vi "GUI_Bella_LaserTable.vi"() -> ()   [LabVIEW 2020]
uses:
  Shared/GUI_Template/GUI_master/tcp_new_data_event.ctl
  Shared/GUI_Template/GUI_master/tcp new data cluster.ctl
  <vilib>/vision/Image Controls.llb/IMAQ Image.ctl
  <vilib>/ErrorRing/Error Ring.xnode
panel:
  in  "Color 8":u32(colorbox) caption="Color"
  in  "Color 7":u32(colorbox) caption="Color"
  in  "Color 6":u32(colorbox)
  in  "Color 5":u32(colorbox) caption="Color"
  in  "Color 4":u32(colorbox) caption="Color"
  in  "Color 3":u32(colorbox) caption="Color"
  in  "Color 2":u32(colorbox) caption="Color"
  in  "Color1":u32(colorbox) caption="Color"
  in  "Color":u32(colorbox)
  in  "size3Y":dbl=280.0 caption="Size Y" min=0.0 max=0.0
  in  "analysis::6":bool caption="Blank Button"
  in  "meancounts::6":dbl=0.001 caption="MeanCounts" min=0.0 max=999999999.0 format="%_4f"
  in  "meancounts::8":dbl=0.001 caption="MeanCounts" min=0.0 max=999999999.0 format="%_4f"
  in  "analysis::8":bool caption="Blank Button"
  in  "size8Y":dbl=125.0 caption="Size Y" min=0.0 max=0.0
  in  "size1Y":dbl=70.0 caption="Size Y" min=0.0 max=0.0
  out "Display8":T1(plugin-control) caption="M1 Cam"
  in  "Target.X::8":dbl=0.001 caption="X" min=0.0 max=2000.0
  in  "Target.Y::8":dbl=0.001 caption="Y" min=0.0 max=2000.0
  in  "size8X":dbl=170.0 caption="Size X" min=0.0 max=0.0
  out "Display7":T1(plugin-control) caption="M1 Cam"
  in  "Target.X::7":dbl=0.001 caption="X" min=0.0 max=2000.0
  in  "Target.Y::7":dbl=0.001 caption="Y" min=0.0 max=2000.0
  in  "size7":dbl=210.0 caption="Size" min=0.0 max=0.0
  out "Display6":T1(plugin-control) caption="M1 Cam"
  in  "Target.X::6":dbl=0.001 caption="X" min=0.0 max=2000.0
  in  "Target.Y::6":dbl=0.001 caption="Y" min=0.0 max=2000.0
  in  "size6":dbl=20.0 caption="Size" min=0.0 max=0.0
  out "error out":errorcluster
  in  "GUIdevice 7":string="CAM-1BL-DM" caption="CAMERA 7"
  in  "GUIdevice 6":string="CAM-LT-Amp3Leak" caption="CAMERA 6"
  in  "GUIdevice 8":string="CAM-1BL-ShotControl" caption="CAMERA 8"
  out "image::7":T1(plugin-control) caption="M1 Cam"
  out "image::8":T1(plugin-control) caption="M1 Cam"
  in  "centroidx::6":dbl=0.001 caption="X" min=0.0 max=0.0
  in  "centroidy::7":dbl=0.001 caption="Y" min=0.0 max=0.0
  in  "centroidx::7":dbl=0.001 caption="X" min=0.0 max=0.0
  in  "exposure::7":dbl=0.001 caption="Exposure" min=3.8e-05 max=1.0 format="%_4p"
  in  "trigger::7":bool caption="Blank Button"
  in  "centroidy::6":dbl=0.001 caption="Y" min=0.0 max=0.0
  in  "exposure::8":dbl=0.001 caption="Exposure" min=3.8e-05 max=1.0 format="%_4p"
  in  "trigger::8":bool caption="Blank Button"
  in  "centroidy::8":dbl=0.001 caption="Y" min=0.0 max=0.0
  in  "centroidx::8":dbl=0.001 caption="X" min=0.0 max=0.0
  in  "exposure::6":dbl=0.001 caption="Exposure" min=3.8e-05 max=1.0 format="%_4p"
  in  "trigger::6":bool caption="Blank Button"
  in  "image::6":T1(plugin-control) caption="M1 Cam"
  in  "roi::6":bool caption="Blank Button"
  in  "roi::7":bool caption="Blank Button"
  in  "roi::8":bool caption="Blank Button"
  out "Display5":T1(plugin-control) caption="M1 Cam"
  in  "Target.X::5":dbl=0.001 caption="X" min=0.0 max=2000.0
  in  "Target.Y::5":dbl=0.001 caption="Y" min=0.0 max=2000.0
  in  "size5":dbl=20.0 caption="Size" min=0.0 max=0.0
  out "Display4":T1(plugin-control) caption="M1 Cam"
  in  "Target.X::4":dbl=0.001 caption="X" min=0.0 max=2000.0
  in  "Target.Y::4":dbl=0.001 caption="Y" min=0.0 max=2000.0
  in  "size4":dbl=20.0 caption="Size" min=0.0 max=0.0
  out "Display3":T1(plugin-control) caption="M1 Cam"
  in  "Target.X::3":dbl=0.001 caption="X" min=0.0 max=2000.0
  in  "Target.Y::3":dbl=0.001 caption="Y" min=0.0 max=2000.0
  in  "size3X":dbl=246.0 caption="Size X" min=0.0 max=0.0
  in  "Target.X::2":dbl=0.001 caption="X" min=0.0 max=2000.0
  in  "Target.Y::2":dbl=0.001 caption="Y" min=0.0 max=2000.0
  in  "size2":dbl=100.0 caption="Size" min=0.0 max=0.0
  out "Display2":T1(plugin-control) caption="M1 Cam"
  in  "roi::5":bool caption="Blank Button"
  in  "centroidx::5":dbl=0.001 caption="X" min=0.0 max=0.0
  in  "centroidy::5":dbl=0.001 caption="Y" min=0.0 max=0.0
  in  "trigger::5":bool caption="Blank Button"
  in  "exposure::5":dbl=0.001 caption="Exposure" min=3.8e-05 max=1.0 format="%_4p"
  in  "GUIdevice 5":string="CAM-LT-Tel3L1" caption="CAMERA 5"
  in  "roi::4":bool caption="Blank Button"
  in  "centroidx::4":dbl=0.001 caption="X" min=0.0 max=0.0
  in  "centroidy::4":dbl=0.001 caption="Y" min=0.0 max=0.0
  in  "trigger::4":bool caption="Blank Button"
  in  "exposure::4":dbl=0.001 caption="Exposure" min=3.8e-05 max=1.0 format="%_4p"
  in  "GUIdevice 4":string="CAM-LT-AMP2mode" caption="CAMERA 4"
  in  "roi::3":bool caption="Blank Button"
  in  "centroidx::3":dbl=0.001 caption="X" min=0.0 max=0.0
  in  "centroidy::3":dbl=0.001 caption="Y" min=0.0 max=0.0
  in  "trigger::3":bool caption="Blank Button"
  in  "exposure::3":dbl=0.001 caption="Exposure" min=3.8e-05 max=1.0 format="%_4p"
  in  "GUIdevice 3":string="CAM-LT-Amp1-Pickoff" caption="CAMERA 3"
  in  "roi::1":bool caption="Blank Button"
  in  "size1X":dbl=70.0 caption="Size X" min=0.0 max=0.0
  in  "Target.X::1":dbl=0.001 caption="X" min=0.0 max=2000.0
  in  "Target.Y::1":dbl=0.001 caption="Y" min=0.0 max=2000.0
  in  "centroidx::1":dbl=0.001 caption="X" min=0.0 max=0.0
  in  "centroidy::1":dbl=0.001 caption="Y" min=0.0 max=0.0
  in  "trigger::1":bool caption="Blank Button"
  in  "exposure::1":dbl=0.001 caption="Exposure" min=3.8e-05 max=1.0 format="%_4p"
  in  "GUIdevice 1":string="CAM-LT-XPW" caption="CAMERA 1"
  out "Display1":T1(plugin-control) caption="M1 Cam"
  in  "roi::2":bool caption="Blank Button"
  in  "centroidx::2":dbl=0.001 caption="X" min=0.0 max=0.0
  in  "centroidy::2":dbl=0.001 caption="Y" min=0.0 max=0.0
  in  "trigger::2":bool caption="Blank Button"
  in  "exposure::2":dbl=0.001 caption="Exposure" min=3.8e-05 max=1.0 format="%_4p"
  in  "GUIdevice 2":string="CAM-LT-Preamp" caption="CAMERA 2"
  out "image::5":T1(plugin-control) caption="M1 Cam"
  out "image::4":T1(plugin-control) caption="M1 Cam"
  in  "image::3":T1(plugin-control) caption="M1 Cam"
  out "image::2":T1(plugin-control) caption="M1 Cam"
  out "image::1":T1(plugin-control) caption="M1 Cam"
  out "tcp data event":T2
  in  "stop":bool
  out "error IO 2":errorcluster
  # "LASER TABLE GUI - 1"
  # "Target"
  # "Centroid"
  # "Centroid"
  # "Target"
  # "Target"
  # "Centroid"
  # "Centroid"
  # "Target"
  # "Centroid"
  # "Target"
  # "Target"
  # "Centroid"
  # "Centroid"
  # "Target"
  # "Centroid"
  # "Target"
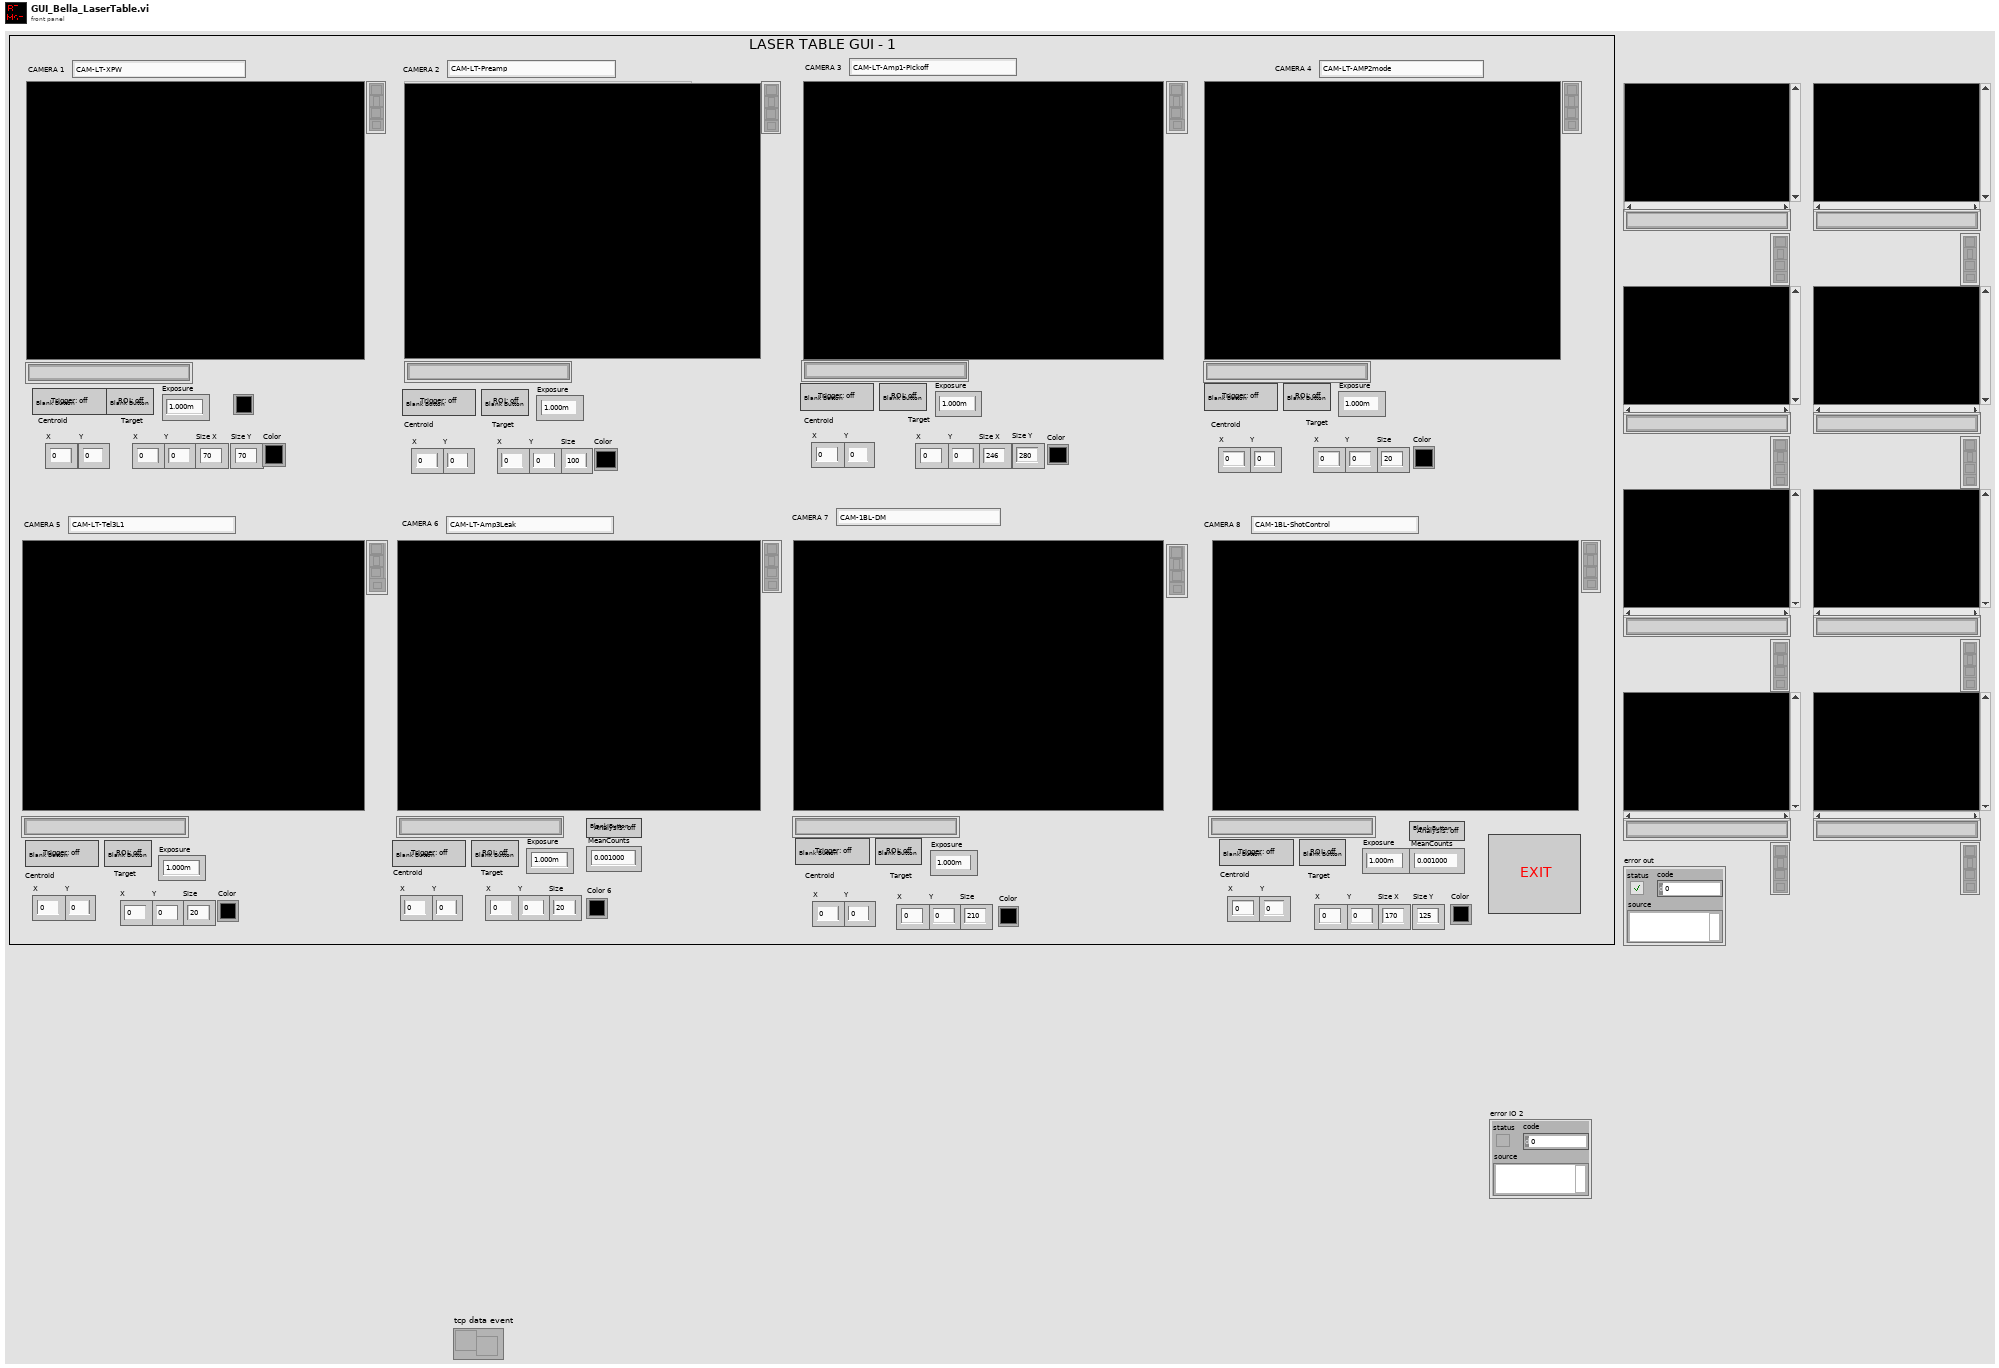
[diagram p1: front panel]
types:
  T1 = typedef "IMAQ Image.ctl" = refnum<image>
  T2 = typedef "tcp_new_data_event.ctl" = refnum<user-event>
  T3 = cluster{"Image1":T1, "Image2":T1, "Image3":T1, "Image4":T1, "Image5":T1, "Image6":T1, "Image7":T1, "Image8":T1}
  T4 = cluster{"Last update Cam1":u32, "Last update Cam2":u32, "Last update Cam3":u32, "Last update Cam4":u32, "Last update Cam5":u32, "Last update Cam6":u32, "Last update Cam7":u32, "Last update Cam8":u32}
  T5 = typedef "Image Type" = u32
  T6 = typedef "tcp new data cluster.ctl" = cluster{"EventEnum":enum16{"new data", "connection status update"}, "Device name":string}
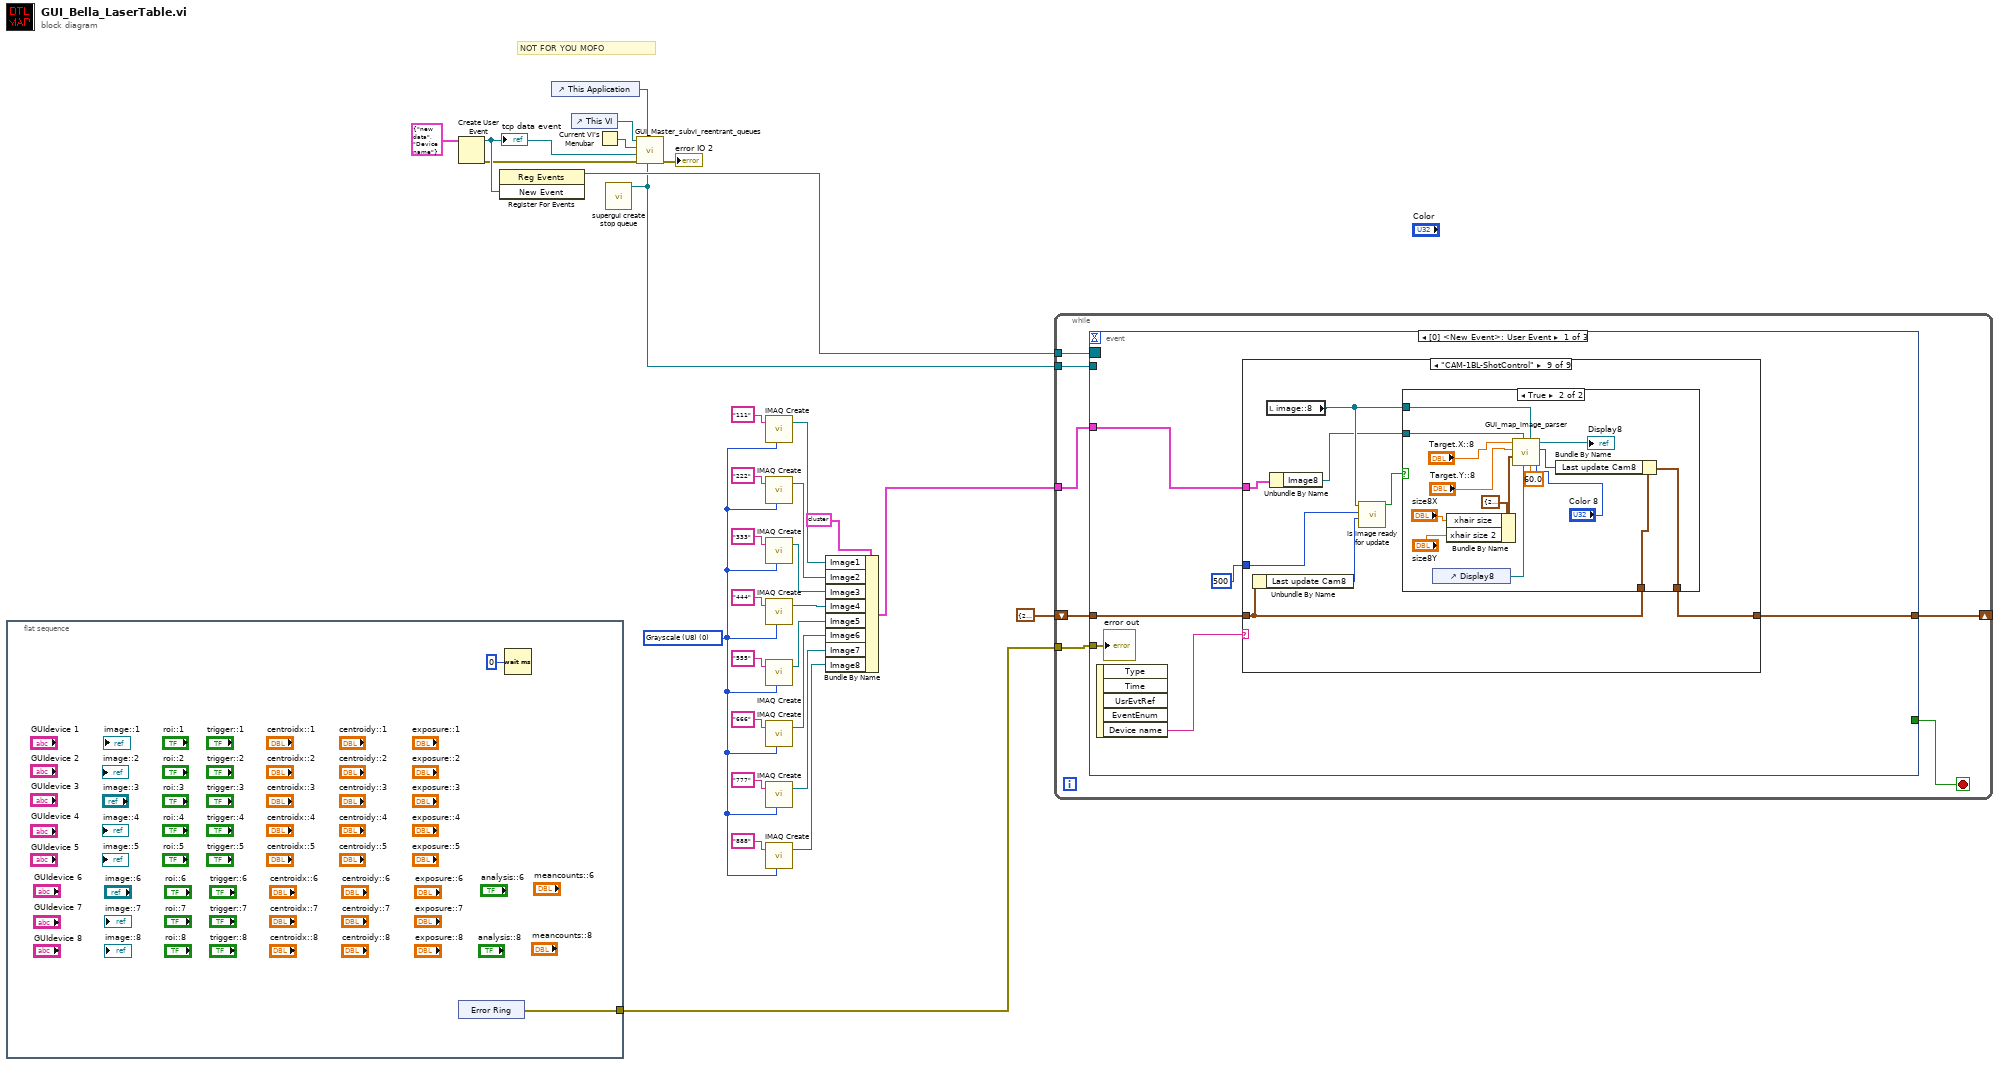
[diagram p0: block diagram]
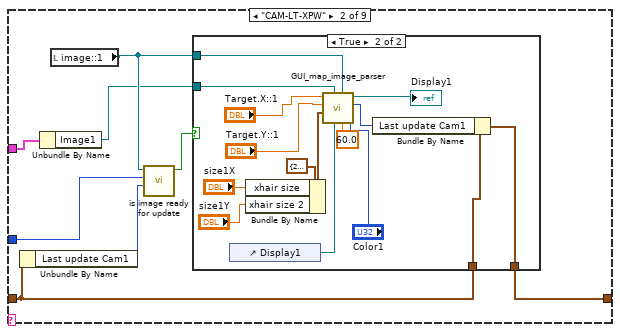
[diagram p3: hidden frame]
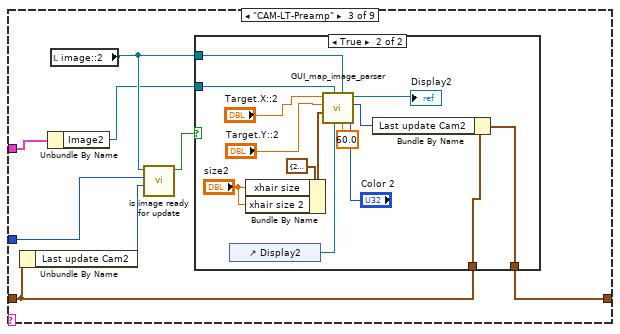
[diagram p5: hidden frame]
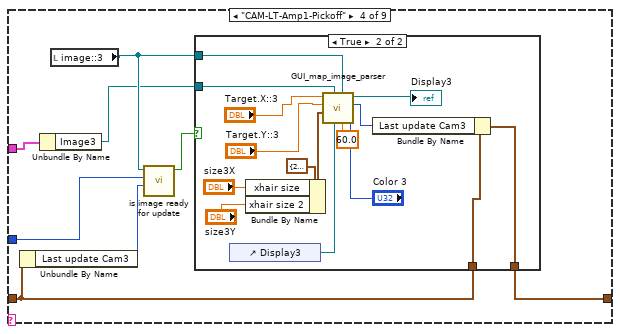
[diagram p7: hidden frame]
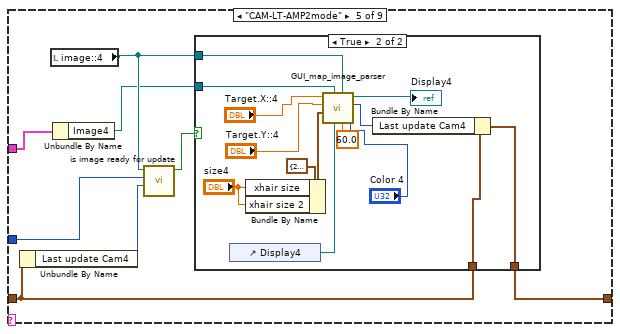
[diagram p9: hidden frame]
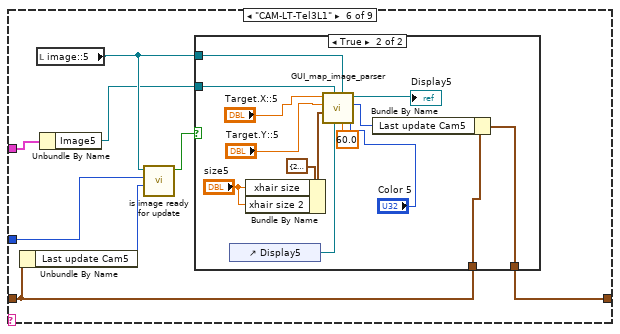
[diagram p11: hidden frame]
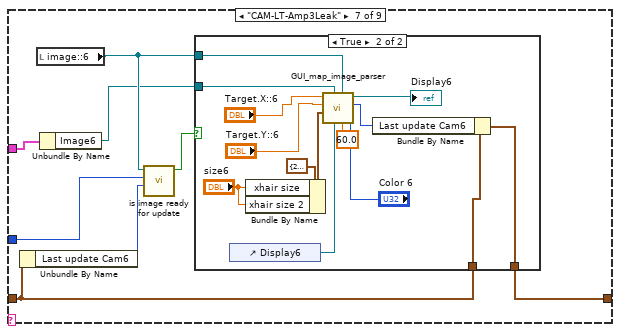
[diagram p13: hidden frame]
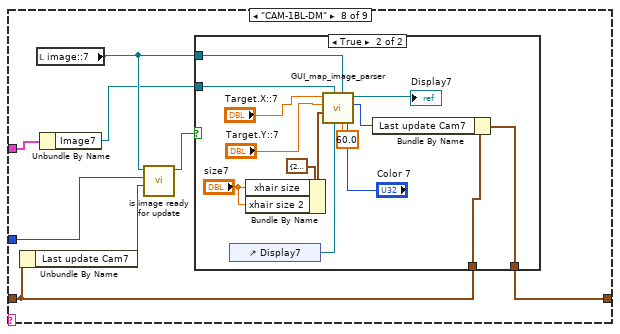
[diagram p15: hidden frame]
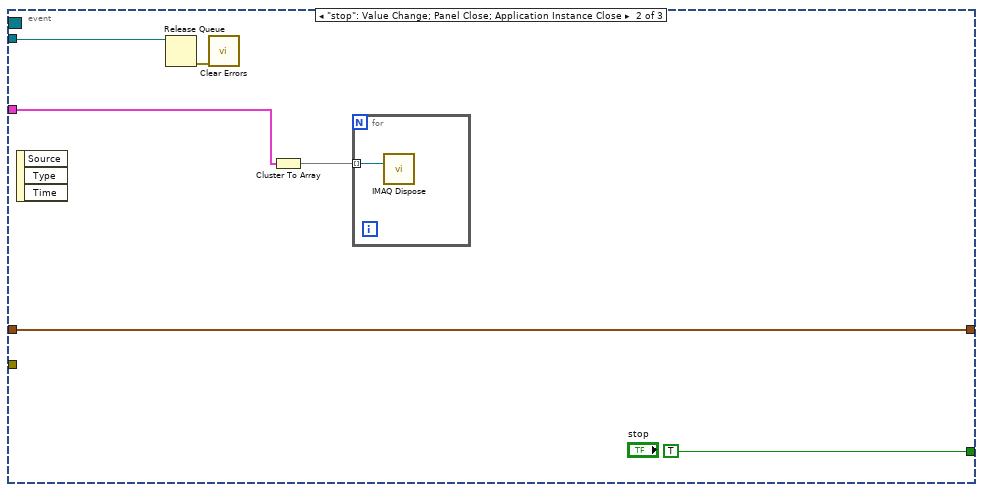
[diagram p18: hidden frame]
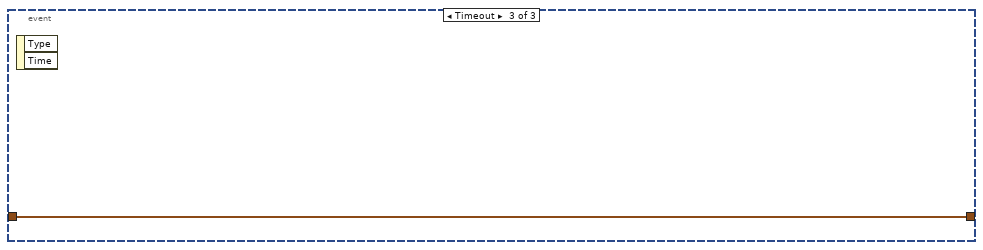
[diagram p19: hidden frame]
diagram:
  w12 = T5 0 items=["Grayscale (U8)", "Grayscale (I16)", "Grayscale (SGL)", "Complex (CSG)", "RGB (U32)", "HSL (U32)", "RGB (U64)", "Grayscale (U16)"] ("Image Type")
  # "NOT FOR YOU MOFO"
  n1 = flat-sequence {
    tunnel: [w32] -> w1
    frame #0 {
      n2 = xnode "Error Ring"() -> ("error out"=w32:errorcluster)
      n3 = Wait (ms)(milliseconds to wait=u32 0) -> ()  [unwired: 1 out]
    }
  }
  n4 = Create User Event(user event datatype=T6 {"EventEnum"=enum."new data", "Device name"="Device name"} ("New Event")) -> (user event=w29:refnum<user-event>, error out=w28:errorcluster)  [unwired: 1 in]
  "tcp data event" <- w29
  n5 = register-events(w29) -> (reference out=w24:refnum<event-registration>)  [unwired: 2 in, 1 out]
  n6 = control-ref of="This Application"() -> (w30:refnum<vi>)
  n7 = control-ref of="This VI"() -> (w25:refnum<vi>)
  n8 = Current VI's Menubar() -> (w26:refnum<k9>)
  n9 = call "supergui create stop queue.vi"() -> ("STOP Queue out"=w16:refnum<queue>)  [unwired: 11 in]
  n10 = call "GUI_Master_subvi_reentrant_queues.vi"("STOP Queue in"=w16, "This Application"=w30, "error in (no error)"=w28, "tcp data event"=w29, "Caller menu reference"=w26, "Caller VI ref"=w25) -> ("error out"=→"error IO 2":errorcluster)  [unwired: 5 in]
  n11 = call "IMAQ Create"("Image Name"="111", "Image Type"=w12) -> ("New Image"=w11:T1)  [unwired: 3 in, 1 out]
  n12 = call "IMAQ Create"("Image Name"="222", "Image Type"=w12) -> ("New Image"=w10:T1)  [unwired: 3 in, 1 out]
  n13 = call "IMAQ Create"("Image Name"="333", "Image Type"=w12) -> ("New Image"=w9:T1)  [unwired: 3 in, 1 out]
  n14 = call "IMAQ Create"("Image Name"="444", "Image Type"=w12) -> ("New Image"=w8:T1)  [unwired: 3 in, 1 out]
  n15 = call "IMAQ Create"("Image Name"="555", "Image Type"=w12) -> ("New Image"=w7:T1)  [unwired: 3 in, 1 out]
  n16 = call "IMAQ Create"("Image Name"="666", "Image Type"=w12) -> ("New Image"=w6:T1)  [unwired: 3 in, 1 out]
  n17 = call "IMAQ Create"("Image Name"="777", "Image Type"=w12) -> ("New Image"=w5:T1)  [unwired: 3 in, 1 out]
  n18 = call "IMAQ Create"("Image Name"="888", "Image Type"=w12) -> ("New Image"=w4:T1)  [unwired: 3 in, 1 out]
  n19 = Bundle By Name(cluster=T3 {"Image1"=refnum, "Image2"=refnum, "Image3"=refnum, "Image4"=refnum, "Image5"=refnum, "Image6"=refnum, "Image7"=refnum, "Image8"=refnum}, "Image1"=w11, "Image2"=w10, "Image3"=w9, "Image4"=w8, "Image5"=w7, "Image6"=w6, "Image7"=w5, "Image8"=w4) -> (w2:T3)
  n20 = while {
    tunnel: w24 -> [w39]
    shift-right: [w37] -> _
    shift-left: T4 {"Last update Cam1"=200, "Last update Cam2"=200, "Last update Cam3"=200, "Last update Cam4"=200, "Last update Cam5"=200, "Last update Cam6"=200, "Last update Cam7"=200, "Last update Cam8"=200} -> [w38]
    tunnel: w16 -> [w36]
    tunnel: w2 -> [w35]
    tunnel: w1 -> [w34]
    stop <- w40 stop-if-true
    n21 = event shown="[0] <New Event>: User Event" {
      selector: w39 -> [_ _ _]
      dyn-events: _ -> [_ _ _]
      timeout: _ -> [_ _ _]
      tunnel: [_ TRUE ("stop") _] -> w40
      tunnel: w38 -> [w45 w239 w242]
      tunnel: [w43 w239 w242] -> w37
      tunnel: w36 -> [_ w238 _]
      tunnel: w35 -> [w42 w236 _]
      tunnel: w34 -> [w41 _ _]
      event User Event {
        n22 = event-data() -> ("Device name"=w46:string)  [unwired: 1 in, 4 out]
        n23 = case shown="\"CAM-1BL-ShotControl\"" w46 {
          tunnel: w45 -> [w47 w55 w79 w102 w126 w149 w172 w195 w218]
          tunnel: u32 500 ("x-y") -> [_ w53 w77 w100 w124 w147 w170 w193 w216]
          tunnel: [w47 w54 w78 w101 w125 w148 w171 w194 w217] -> w43
          tunnel: w42 -> [_ w49 w73 w96 w120 w143 w166 w189 w212]
          frame Default {
          }
          frame "CAM-LT-XPW" {
            n24 = Unbundle By Name(w55) -> ("Last update Cam1"=w52:u32)
            n25 = Unbundle By Name(w49) -> ("Image1"=w48:T1)
            n26 = local read "image::1"() -> (w50:T1)
            n27 = call "is image ready for update.vi"("Last update"=w52, "min time between updates"=w53, "image ref in"=w50) -> ("update image"=w51:bool)  [unwired: 8 in]
            n28 = case shown="True" w51 {
              tunnel: w55 -> [w56 w71]
              tunnel: [w56 w70] -> w54
              tunnel: w50 -> [_ w69]
              tunnel: w48 -> [_ w59]
              frame False {
              }
              frame True {
                n29 = control-ref of="Display1"() -> (w65:refnum<vi>)
                n30 = Bundle By Name(cluster=cluster{"xhair size":dbl, "xhair size 2":dbl} {"xhair size"=20.0, "xhair size 2"=20.0} ("size"), "xhair size"="size1X", "xhair size 2"="size1Y") -> (w60:cluster{"xhair size":dbl, "xhair size 2":dbl})
                n31 = call "GUI_map_image_parser.vi"("color"="Color1", "zoom#"=60.0, "Image Src"=w69, "Ctl Refnum"=w65, "Image Dst"=w59, "size"=w60, "target y"="Target.Y::1", "target x"="Target.X::1") -> ("ms timer out"=w64:u32, "Img out"=→"Display1":T1)  [unwired: 2 in]
                n32 = Bundle By Name(cluster=w71, "Last update Cam1"=w64) -> (w70:T4)
              }
            }
          }
          frame "CAM-LT-Preamp" {
            n33 = Unbundle By Name(w79) -> ("Last update Cam2"=w76:u32)
            n34 = Unbundle By Name(w73) -> ("Image2"=w72:T1)
            n35 = local read "image::2"() -> (w74:T1)
            n36 = call "is image ready for update.vi"("Last update"=w76, "min time between updates"=w77, "image ref in"=w74) -> ("update image"=w75:bool)  [unwired: 8 in]
            n37 = case shown="True" w75 {
              tunnel: w79 -> [w80 w94]
              tunnel: [w80 w93] -> w78
              tunnel: w74 -> [_ w92]
              tunnel: w72 -> [_ w82]
              frame False {
              }
              frame True {
                n38 = control-ref of="Display2"() -> (w88:refnum<vi>)
                n39 = Bundle By Name(cluster=cluster{"xhair size":dbl, "xhair size 2":dbl} {"xhair size"=20.0, "xhair size 2"=20.0} ("size"), "xhair size"="size2", "xhair size 2"="size2") -> (w83:cluster{"xhair size":dbl, "xhair size 2":dbl})
                n40 = call "GUI_map_image_parser.vi"("color"="Color 2", "zoom#"=60.0, "Image Src"=w92, "Ctl Refnum"=w88, "Image Dst"=w82, "size"=w83, "target y"="Target.Y::2", "target x"="Target.X::2") -> ("ms timer out"=w87:u32, "Img out"=→"Display2":T1)  [unwired: 2 in]
                n41 = Bundle By Name(cluster=w94, "Last update Cam2"=w87) -> (w93:T4)
              }
            }
          }
          frame "CAM-LT-Amp1-Pickoff" {
            n42 = Unbundle By Name(w102) -> ("Last update Cam3"=w99:u32)
            n43 = Unbundle By Name(w96) -> ("Image3"=w95:T1)
            n44 = local read "image::3"() -> (w97:T1)
            n45 = call "is image ready for update.vi"("Last update"=w99, "min time between updates"=w100, "image ref in"=w97) -> ("update image"=w98:bool)  [unwired: 8 in]
            n46 = case shown="True" w98 {
              tunnel: w102 -> [w103 w118]
              tunnel: [w103 w117] -> w101
              tunnel: w97 -> [_ w116]
              tunnel: w95 -> [_ w106]
              frame False {
              }
              frame True {
                n47 = control-ref of="Display3"() -> (w112:refnum<vi>)
                n48 = Bundle By Name(cluster=cluster{"xhair size":dbl, "xhair size 2":dbl} {"xhair size"=20.0, "xhair size 2"=20.0} ("size"), "xhair size"="size3X", "xhair size 2"="size3Y") -> (w107:cluster{"xhair size":dbl, "xhair size 2":dbl})
                n49 = call "GUI_map_image_parser.vi"("color"="Color 3", "zoom#"=60.0, "Image Src"=w116, "Ctl Refnum"=w112, "Image Dst"=w106, "size"=w107, "target y"="Target.Y::3", "target x"="Target.X::3") -> ("ms timer out"=w111:u32, "Img out"=→"Display3":T1)  [unwired: 2 in]
                n50 = Bundle By Name(cluster=w118, "Last update Cam3"=w111) -> (w117:T4)
              }
            }
          }
          frame "CAM-LT-AMP2mode" {
            n51 = Unbundle By Name(w126) -> ("Last update Cam4"=w123:u32)
            n52 = local read "image::4"() -> (w121:T1)
            n53 = Unbundle By Name(w120) -> ("Image4"=w119:T1)
            n54 = call "is image ready for update.vi"("Last update"=w123, "min time between updates"=w124, "image ref in"=w121) -> ("update image"=w122:bool)  [unwired: 8 in]
            n55 = case shown="True" w122 {
              tunnel: w126 -> [w127 w141]
              tunnel: [w127 w140] -> w125
              tunnel: w121 -> [_ w139]
              tunnel: w119 -> [_ w129]
              frame False {
              }
              frame True {
                n56 = control-ref of="Display4"() -> (w135:refnum<vi>)
                n57 = Bundle By Name(cluster=cluster{"xhair size":dbl, "xhair size 2":dbl} {"xhair size"=20.0, "xhair size 2"=20.0} ("size"), "xhair size"="size4", "xhair size 2"="size4") -> (w130:cluster{"xhair size":dbl, "xhair size 2":dbl})
                n58 = call "GUI_map_image_parser.vi"("color"="Color 4", "zoom#"=60.0, "Image Src"=w139, "Ctl Refnum"=w135, "Image Dst"=w129, "size"=w130, "target y"="Target.Y::4", "target x"="Target.X::4") -> ("ms timer out"=w134:u32, "Img out"=→"Display4":T1)  [unwired: 2 in]
                n59 = Bundle By Name(cluster=w141, "Last update Cam4"=w134) -> (w140:T4)
              }
            }
          }
          frame "CAM-LT-Tel3L1" {
            n60 = Unbundle By Name(w149) -> ("Last update Cam5"=w146:u32)
            n61 = local read "image::5"() -> (w144:T1)
            n62 = Unbundle By Name(w143) -> ("Image5"=w142:T1)
            n63 = call "is image ready for update.vi"("Last update"=w146, "min time between updates"=w147, "image ref in"=w144) -> ("update image"=w145:bool)  [unwired: 8 in]
            n64 = case shown="True" w145 {
              tunnel: w149 -> [w150 w164]
              tunnel: [w150 w163] -> w148
              tunnel: w144 -> [_ w162]
              tunnel: w142 -> [_ w152]
              frame False {
              }
              frame True {
                n65 = control-ref of="Display5"() -> (w158:refnum<vi>)
                n66 = Bundle By Name(cluster=cluster{"xhair size":dbl, "xhair size 2":dbl} {"xhair size"=20.0, "xhair size 2"=20.0} ("size"), "xhair size"="size5", "xhair size 2"="size5") -> (w153:cluster{"xhair size":dbl, "xhair size 2":dbl})
                n67 = call "GUI_map_image_parser.vi"("color"="Color 5", "zoom#"=60.0, "Image Src"=w162, "Ctl Refnum"=w158, "Image Dst"=w152, "size"=w153, "target y"="Target.Y::5", "target x"="Target.X::5") -> ("ms timer out"=w157:u32, "Img out"=→"Display5":T1)  [unwired: 2 in]
                n68 = Bundle By Name(cluster=w164, "Last update Cam5"=w157) -> (w163:T4)
              }
            }
          }
          frame "CAM-LT-Amp3Leak" {
            n69 = Unbundle By Name(w172) -> ("Last update Cam6"=w169:u32)
            n70 = local read "image::6"() -> (w167:T1)
            n71 = Unbundle By Name(w166) -> ("Image6"=w165:T1)
            n72 = call "is image ready for update.vi"("Last update"=w169, "min time between updates"=w170, "image ref in"=w167) -> ("update image"=w168:bool)  [unwired: 8 in]
            n73 = case shown="True" w168 {
              tunnel: w172 -> [w173 w187]
              tunnel: [w173 w186] -> w171
              tunnel: w167 -> [_ w185]
              tunnel: w165 -> [_ w175]
              frame False {
              }
              frame True {
                n74 = control-ref of="Display6"() -> (w181:refnum<vi>)
                n75 = Bundle By Name(cluster=cluster{"xhair size":dbl, "xhair size 2":dbl} {"xhair size"=20.0, "xhair size 2"=20.0} ("size"), "xhair size"="size6", "xhair size 2"="size6") -> (w176:cluster{"xhair size":dbl, "xhair size 2":dbl})
                n76 = call "GUI_map_image_parser.vi"("color"="Color 6", "zoom#"=60.0, "Image Src"=w185, "Ctl Refnum"=w181, "Image Dst"=w175, "size"=w176, "target y"="Target.Y::6", "target x"="Target.X::6") -> ("ms timer out"=w180:u32, "Img out"=→"Display6":T1)  [unwired: 2 in]
                n77 = Bundle By Name(cluster=w187, "Last update Cam6"=w180) -> (w186:T4)
              }
            }
          }
          frame "CAM-1BL-DM" {
            n78 = Unbundle By Name(w195) -> ("Last update Cam7"=w192:u32)
            n79 = local read "image::7"() -> (w190:T1)
            n80 = Unbundle By Name(w189) -> ("Image7"=w188:T1)
            n81 = call "is image ready for update.vi"("Last update"=w192, "min time between updates"=w193, "image ref in"=w190) -> ("update image"=w191:bool)  [unwired: 8 in]
            n82 = case shown="True" w191 {
              tunnel: w195 -> [w196 w210]
              tunnel: [w196 w209] -> w194
              tunnel: w190 -> [_ w208]
              tunnel: w188 -> [_ w198]
              frame False {
              }
              frame True {
                n83 = control-ref of="Display7"() -> (w204:refnum<vi>)
                n84 = Bundle By Name(cluster=cluster{"xhair size":dbl, "xhair size 2":dbl} {"xhair size"=20.0, "xhair size 2"=20.0} ("size"), "xhair size"="size7", "xhair size 2"="size7") -> (w199:cluster{"xhair size":dbl, "xhair size 2":dbl})
                n85 = call "GUI_map_image_parser.vi"("color"="Color 7", "zoom#"=60.0, "Image Src"=w208, "Ctl Refnum"=w204, "Image Dst"=w198, "size"=w199, "target y"="Target.Y::7", "target x"="Target.X::7") -> ("ms timer out"=w203:u32, "Img out"=→"Display7":T1)  [unwired: 2 in]
                n86 = Bundle By Name(cluster=w210, "Last update Cam7"=w203) -> (w209:T4)
              }
            }
          }
          frame "CAM-1BL-ShotControl" {
            n87 = Unbundle By Name(w218) -> ("Last update Cam8"=w215:u32)
            n88 = local read "image::8"() -> (w213:T1)
            n89 = Unbundle By Name(w212) -> ("Image8"=w211:T1)
            n90 = call "is image ready for update.vi"("Last update"=w215, "min time between updates"=w216, "image ref in"=w213) -> ("update image"=w214:bool)  [unwired: 8 in]
            n91 = case shown="True" w214 {
              tunnel: w218 -> [w219 w234]
              tunnel: [w219 w233] -> w217
              tunnel: w213 -> [_ w232]
              tunnel: w211 -> [_ w222]
              frame False {
              }
              frame True {
                n92 = control-ref of="Display8"() -> (w228:refnum<vi>)
                n93 = Bundle By Name(cluster=cluster{"xhair size":dbl, "xhair size 2":dbl} {"xhair size"=20.0, "xhair size 2"=20.0} ("size"), "xhair size"="size8X", "xhair size 2"="size8Y") -> (w223:cluster{"xhair size":dbl, "xhair size 2":dbl})
                n94 = call "GUI_map_image_parser.vi"("color"="Color 8", "zoom#"=60.0, "Image Src"=w232, "Ctl Refnum"=w228, "Image Dst"=w222, "size"=w223, "target y"="Target.Y::8", "target x"="Target.X::8") -> ("ms timer out"=w227:u32, "Img out"=→"Display8":T1)  [unwired: 2 in]
                n95 = Bundle By Name(cluster=w234, "Last update Cam8"=w227) -> (w233:T4)
              }
            }
          }
        }
        "error out" <- w41
      }
      event "stop": Value Change; Panel Close; Application Instance Close {
        n96 = event-data() -> ()  [unwired: 1 in, 3 out]
        n97 = Release Queue(queue=w238) -> (error out=w237:errorcluster)  [unwired: 2 in, 2 out]
        n98 = call <vilib>:"Clear Errors.vi"("error in (no error)"=w237) -> ()  [unwired: 5 in, 2 out]
        n99 = Cluster To Array(cluster=w236) -> (array=w235:T1[])
        n100 = for {
          tunnel: w235 -> [w241] mode=indexing
          n101 = call "IMAQ Dispose"("Image"=w241) -> ()  [unwired: 5 in, 1 out]
        }
      }
      event Timeout {
        n102 = event-data() -> ()  [unwired: 1 in, 2 out]
      }
    }
  }
